vi "NR Call Handover.vi"(8 "error in (no error)":errorcluster caption="에러 입력(에러 없음)", 10 "NR Call Handover Param":T1, 11 "Instrument Manager 입력":refnum<class "Instrument Manager.lvclass">) -> (0 "error out":errorcluster caption="에러 출력", 3 "Instrument Manager 출력":refnum<class "Instrument Manager.lvclass">)   [LabVIEW 2023, in "Instrument Manager.lvclass"]
uses:
  Instrument Manager.lvclass
  Type Definition/NR Call Handover Param.ctl
  Module/ANRITSU Call Box/Type Definition/NR Modulation Type.ctl
  Instrument Manager.lvclass/Instrument Manager.ctl
  Module/ANRITSU Call Box/ANRITSU Call Box.lvlib
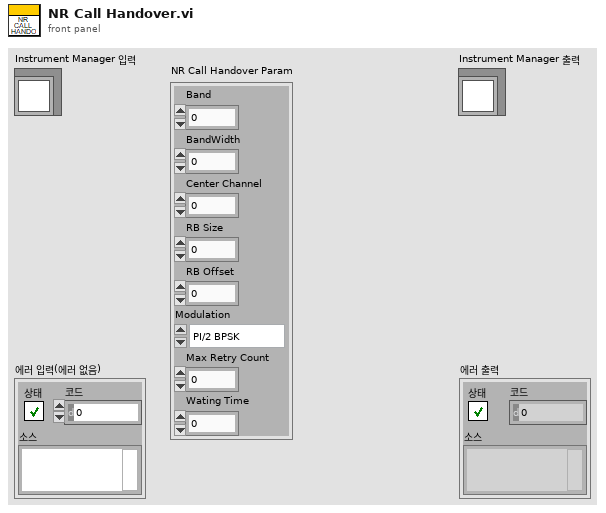
[diagram p1: front panel]
types:
  T1 = typedef "NR Call Handover Param.ctl" = cluster{"Band":u32, "BandWidth":u32, "Center Channel":u32, "RB Size":i32, "RB Offset":i32, "Modulation":T2, "Max Retry Count":i32, "Wating Time":i32}
  T2 = typedef "ANRITSU Call Box.lvlib/NR Modulation Type.ctl" = enum16{"PI/2 BPSK", "QPSK", "16QAM", "64QAM", "256QAM"}
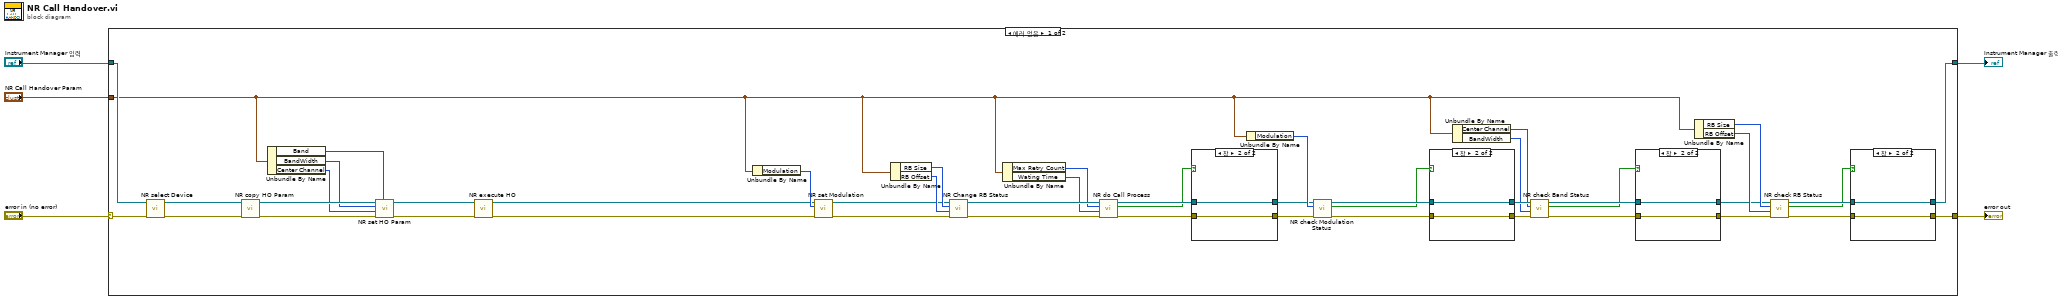
[diagram p0: block diagram]
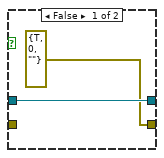
[diagram p2: hidden frame]
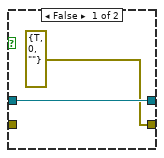
[diagram p3: hidden frame]
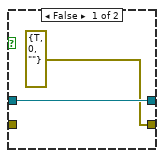
[diagram p4: hidden frame]
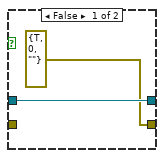
[diagram p5: hidden frame]
diagram:
  n1 = case shown="에러 없음" "error in (no error)" {
    selector: "error in (no error)" -> [w21 w71]
    tunnel: [w42 w71] -> w1
    tunnel: [w41 w70] -> w2
    tunnel: "Instrument Manager 입력" -> [w20 w70]
    tunnel: "NR Call Handover Param" -> [w17 _]
    frame No Error {
      n2 = call "NR select Device.vi"("error in (no error)"=w21, "Instrument Manager 입력"=w20) -> ("error out"=w15:errorcluster, "Instrument Manager 출력"=w16:refnum<class "Instrument Manager.lvclass">)  [unwired: 8 in]
      n3 = call "NR copy HO Param.vi"("error in (no error)"=w15, "Instrument Manager 입력"=w16) -> ("error out"=w13:errorcluster, "Instrument Manager 출력"=w14:refnum<class "Instrument Manager.lvclass">)  [unwired: 8 in]
      n4 = Unbundle By Name(w17) -> ("Band"=w12:u32, "BandWidth"=w11:u32, "Center Channel"=w10:u32)
      n5 = call "NR set HO Param.vi"("Operation Band"=w12, "error in (no error)"=w13, "Center Channel Number"=w10, "BW (MHz)"=w11, "Instrument Manager 입력"=w14) -> ("error out"=w8:errorcluster, "Instrument Manager 출력"=w9:refnum<class "Instrument Manager.lvclass">)  [unwired: 5 in]
      n6 = call "NR execute HO.vi"("error in (no error)"=w8, "Instrument Manager 입력"=w9) -> ("error out"=w7:errorcluster, "Instrument Manager 출력"=w6:refnum<class "Instrument Manager.lvclass">)  [unwired: 8 in]
      n7 = Unbundle By Name(w17) -> ("Modulation"=w24:T2)
      n8 = call "NR set Modulation.vi"("error in (no error)"=w7, "Modulation"=w24, "Instrument Manager 입력"=w6) -> ("error out"=w19:errorcluster, "Instrument Manager 출력"=w18:refnum<class "Instrument Manager.lvclass">)  [unwired: 7 in]
      n9 = Unbundle By Name(w17) -> ("RB Size"=w35:i32, "RB Offset"=w34:i32)
      n10 = call "NR Change RB Status.vi"("error in (no error)"=w19, "RB Offset"=w34, "RB Size"=w35, "Instrument Manager 입력"=w18) -> ("error out"=w29:errorcluster, "Instrument Manager 출력"=w27:refnum<class "Instrument Manager.lvclass">)  [unwired: 6 in]
      n11 = Unbundle By Name(w17) -> ("Max Retry Count"=w22:i32, "Wating Time"=w23:i32)
      n12 = call "NR do Call Process.vi"("error in (no error)"=w29, "Waiting Time"=w23, "Max Retry Count"=w22, "Instrument Manager 입력"=w27) -> ("error out"=w28:errorcluster, "Connected?"=w25:bool, "Instrument Manager 출력"=w26:refnum<class "Instrument Manager.lvclass">)  [unwired: 5 in]
      n13 = case shown="참" w25 {
        tunnel: w26 -> [w55 w57]
        tunnel: [w55 w57] -> w31
        tunnel: [errorcluster {"status"=TRUE, "code"=0, "source"=""} ("error out") w56] -> w30
        tunnel: w28 -> [_ w56]
        frame False {
        }
        frame True {
        }
      }
      n14 = Unbundle By Name(w17) -> ("Modulation"=w40:T2)
      n15 = call "NR check Modulation Status.vi"("error in (no error)"=w30, "Modulation"=w40, "Instrument Manager 입력"=w31) -> ("error out"=w52:errorcluster, "Success?"=w47:bool, "Instrument Manager 출력"=w53:refnum<class "Instrument Manager.lvclass">)  [unwired: 6 in]
      n16 = case shown="참" w47 {
        tunnel: w53 -> [w67 w69]
        tunnel: [w67 w69] -> w51
        tunnel: [errorcluster {"status"=TRUE, "code"=0, "source"=""} ("error out") w68] -> w50
        tunnel: w52 -> [_ w68]
        frame False {
        }
        frame True {
        }
      }
      n17 = Unbundle By Name(w17) -> ("Center Channel"=w38:u32, "BandWidth"=w39:u32)
      n18 = call "NR check Band Status.vi"("error in (no error)"=w50, "BW (MHz)"=w39, "Center Channel Number"=w38, "Instrument Manager 입력"=w51) -> ("error out"=w49:errorcluster, "Success?"=w46:bool, "Instrument Manager 출력"=w48:refnum<class "Instrument Manager.lvclass">)  [unwired: 5 in]
      n19 = case shown="참" w46 {
        tunnel: w48 -> [w63 w65]
        tunnel: [w63 w65] -> w33
        tunnel: [errorcluster {"status"=TRUE, "code"=0, "source"=""} ("error out") w64] -> w32
        tunnel: w49 -> [_ w64]
        frame False {
        }
        frame True {
        }
      }
      n20 = Unbundle By Name(w17) -> ("RB Size"=w36:i32, "RB Offset"=w37:i32)
      n21 = call "NR check RB Status.vi"("error in (no error)"=w32, "RB Offset"=w37, "RB Size"=w36, "Instrument Manager 입력"=w33) -> ("error out"=w44:errorcluster, "Success?"=w43:bool, "Instrument Manager 출력"=w45:refnum<class "Instrument Manager.lvclass">)  [unwired: 5 in]
      n22 = case shown="참" w43 {
        tunnel: w45 -> [w59 w61]
        tunnel: [w59 w61] -> w41
        tunnel: [errorcluster {"status"=TRUE, "code"=0, "source"=""} ("error out") w60] -> w42
        tunnel: w44 -> [_ w60]
        frame False {
        }
        frame True {
        }
      }
    }
    frame Error {
    }
  }
  "error out" <- w1
  "Instrument Manager 출력" <- w2
